vi "Initialize.vi"(8 "error in (no error)":errorcluster, 10 "parent":string, 11 "test handler in":refnum<class "Test Handler.lvclass">) -> (0 "error out":errorcluster, 2 "name":string, 3 "test handler out":refnum<class "Test Handler.lvclass">)   [LabVIEW 2024, in "Test Handler.lvclass"]
uses:
  Test Handler.lvclass
  Test Handler.lvclass/Test Handler.ctl
  src/api/extension/formatting_handler_interface/Formatting Handler.lvclass
panel:
  # "Connector Pane"
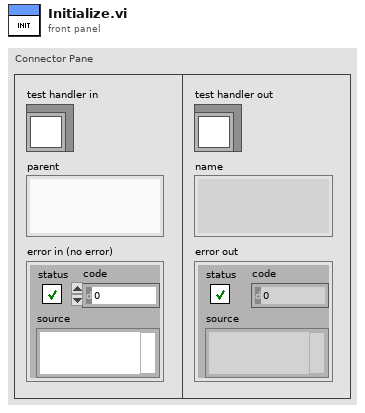
[diagram p1: front panel]
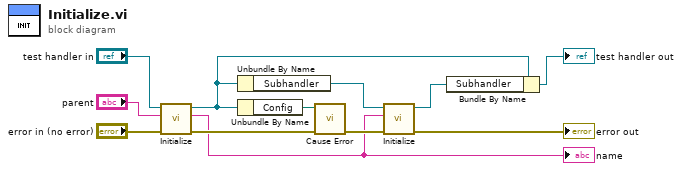
[diagram p0: block diagram]
diagram:
  n1 = call-parent "Initialize.vi"("error in (no error)"="error in (no error)", "logger name"="parent", "handler in"="test handler in") -> ("error out"=w5:errorcluster, "handler name"=w2:string, "handler out"=w3:refnum<class "Test Handler.lvclass">)  [unwired: 6 in]
  "name" <- w2
  n2 = Unbundle By Name(w3) -> ("Subhandler"=w10:refnum<class "Formatting Handler.lvclass">)
  n3 = Unbundle By Name(w3) -> ("Config"=w11:path)
  n4 = call "Cause Error.vi"("error in (no error)"=w5, "ini file path"=w11) -> ("error out"=w7:errorcluster)  [unwired: 8 in, 1 out]
  n5 = call-dynamic "Initialize.vi"("error in (no error)"=w7, "logger name"=w2, "handler in"=w10) -> ("error out"=→"error out":errorcluster, "handler out"=w8:refnum<class "Formatting Handler.lvclass">)  [unwired: 6 in, 1 out]
  n6 = Bundle By Name(cluster=w3, "Subhandler"=w8) -> (→"test handler out":refnum<class "Test Handler.lvclass">)
